vi "EPC300X Utility MODBUS RTU Send Message.vi"(6 "Command (0)":u8, 7 "Unit Address (1)":u8, 8 "error in (no error)":errorcluster, 10 "Message (empty array)":u8[](array[numeric]), 11 "VISA session":refnum<visa-resource-name>) -> (0 "error out":errorcluster, 2 "Length Of Sent MSG":u8, 3 "dup VISA session":refnum<visa-resource-name>)   [LabVIEW 2022 SP3]
doc: "This VI sends the MODBUS message."
panel:
  out "chaine envoyée":string
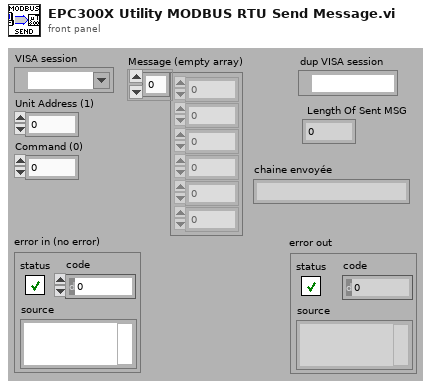
[diagram p1: front panel]
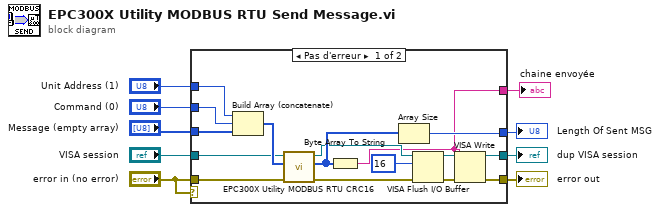
[diagram p0: block diagram]
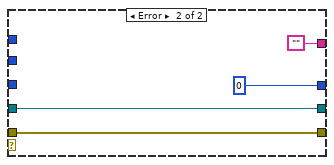
[diagram p2: hidden frame]
diagram:
  n1 = case shown="Pas d'erreur" "error in (no error)" {
    tunnel: "error in (no error)" -> [w25 w28]
    tunnel: [w16 w28] -> w9
    tunnel: [w17 w29] -> w8
    tunnel: "Command (0)" -> [w24 _]
    tunnel: "Unit Address (1)" -> [w23 _]
    tunnel: "VISA session" -> [w21 w29]
    tunnel: [w20 0] -> w4
    tunnel: "Message (empty array)" -> [w18 _]
    tunnel: [w10 ""] -> w1
    frame No Error {
      n2 = Build Array (concatenate)(w23, w24, w18) -> (w22:u8[])
      n3 = call "EPC300X Utility MODBUS RTU CRC16.vi"("error in (no error)"=w25, "Message (empty array)"=w22, "VISA session"=w21) -> ("error out"=w13:errorcluster, "Message with CRC"=w19:u8[], "dup VISA session"=w14:refnum<visa-resource-name>)  [unwired: 5 in, 1 out]
      n4 = Byte Array To String(unsigned byte array=w19) -> (string=w10:string)
      n5 = Array Size(array=w19) -> (size(s)=w20:i32)
      n6 = VISA Flush I/O Buffer(VISA resource name=w14, mask (16)=u16 16, error in (no error)=w13) -> (VISA resource name out=w15:refnum<visa-resource-name>, error out=w12:errorcluster)
      n7 = VISA Write(VISA resource name=w15, write buffer=w10, error in (no error)=w12) -> (VISA resource name out=w17:refnum<visa-resource-name>, error out=w16:errorcluster)  [unwired: 1 out]
    }
    frame Error {
    }
  }
  "error out" <- w9
  "dup VISA session" <- w8
  "Length Of Sent MSG" <- w4
  "chaine envoyée" <- w1
